vi "Project Task Rows.vi"(8 "error in":errorcluster, 10 "Project ID":string, 11 "Project Store in":refnum<class "Project Store.lvclass">) -> (0 "error out":errorcluster, 2 "Task Rows":T1[](array[typedef]), 3 "Project Store out":refnum<class "Project Store.lvclass">)   [LabVIEW 2026]
doc: "Returns every task of one project - active and inactive - in Sort Order, as Task Edit Row clusters {Task Name, Active}, for an editable task list such as the one in New Project.vi. An empty or unknown Project ID gives an empty array and no error. Nothing is written.\n\nInputs: Project Store in (already read from its data source); Project ID; error in.\nOutputs: Project Store out; Task Rows (Sort Order, inactive tasks included); error out.\n\nGenerated by: Claude"
uses:
  Storage/Project Store/Project Store.lvclass
  Task Edit Row.ctl
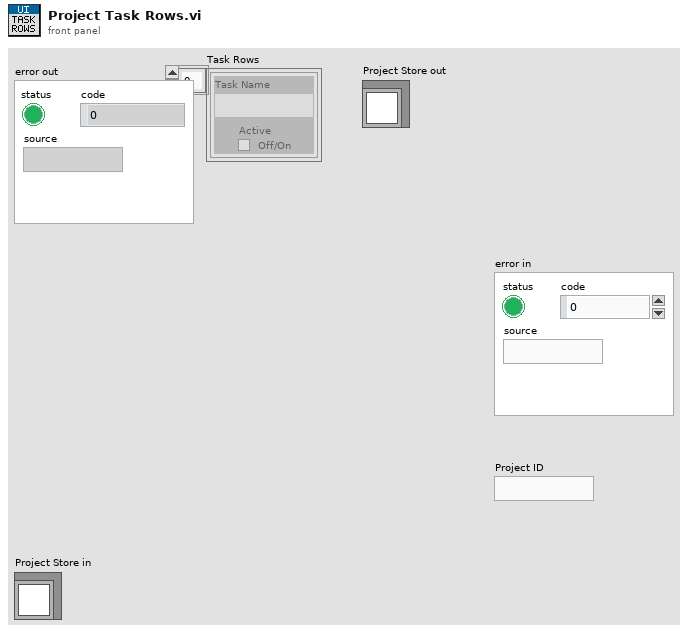
[diagram p1: front panel]
types:
  T1 = typedef "Task Edit Row.ctl" = cluster{"Task Name":string, "Active":bool}
  T2 = typedef "Task List.ctl" = T3[]
  T3 = typedef "Task.ctl" = cluster{"ID":string, "Project ID":string, "Name":string, "Active":bool, "Sort Order":i32}
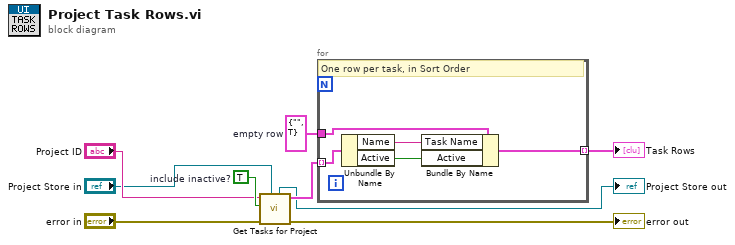
[diagram p0: block diagram]
diagram:
  w8 = T1 {"Task Name"="", "Active"=TRUE}  # empty row
  w7 = TRUE  # include inactive?
  n1 = call-dynamic "Get Tasks for Project.vi"("Project Store in"="Project Store in", "error in (no error)"="error in", "include inactive?"=w7, "Project ID"="Project ID") -> ("error out"=→"error out":errorcluster, "Tasks"=w9:T2, "Project Store out"=→"Project Store out":refnum<class "Project Store.lvclass">)  [unwired: 5 in]
  n2 = for {
    tunnel: w8 -> [w11]
    tunnel: w9 -> [w10] mode=indexing
    tunnel: [w14] -> w5 mode=indexing
    # "One row per task, in Sort Order"
    n3 = Unbundle By Name(w10) -> ("Name"=w12:string, "Active"=w13:bool)
    n4 = Bundle By Name(cluster=w11, "Task Name"=w12, "Active"=w13) -> (w14:T1)
  }
  "Task Rows" <- w5
